vi "Latency Init.vi"() -> (3 "latency metric":T1)   [LabVIEW 2021, in "CAN_Reader_CANsub_Test_Helpers.lvlib"]
uses:
  CAN_Reader_CANsub_Test_Helpers.lvlib
  Latency Metric.ctl
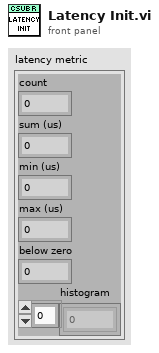
[diagram p1: front panel]
types:
  T1 = typedef "CAN_Reader_CANsub_Test_Helpers.lvlib/Latency Metric.ctl" = cluster{"count":u32, "sum (us)":dbl, "min (us)":dbl, "max (us)":dbl, "below zero":u32, "histogram":u32[]}
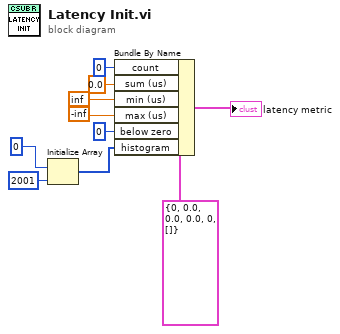
[diagram p0: block diagram]
diagram:
  n1 = Initialize Array(u32 0, 2001 ("dimension size")) -> (w7:u32[])
  n2 = Bundle By Name(cluster=T1 {"count"=0, "sum (us)"=0.0, "min (us)"=0.0, "max (us)"=0.0, "below zero"=0, "histogram"=[]} ("Latency Metric"), "count"=u32 0, "sum (us)"=0.0, "min (us)"=inf, "max (us)"=-inf, "below zero"=u32 0, "histogram"=w7) -> (→"latency metric":T1)
